vi "openDocuement.vi"(8 "error in (no error)":errorcluster, 11 "MS-Word in":refnum<class "MS-Word.lvclass">) -> (0 "error out":errorcluster, 3 "MS-Word out":refnum<class "MS-Word.lvclass">)   [LabVIEW 2017, in "LabVIEW NPOI.lvlib" / "MS-Word.lvclass"]
doc: "Protected dynamic dispatch method to open the <b>Document</b> file located at <b>File Path</b> for reading."
uses:
  MS-Word.lvclass
  C:/Users/Neo/Desktop/Dev_Tools_BR/LabVIEW_NPOI/src/LabVIEW NPOI/Document/Document.lvclass
  Document/Document.lvclass/Document.ctl
  MS-Word.lvclass/MS-Word.ctl
  Document/Get FilePath.vi
  xwpfDocument/xwpfDocument.lvclass
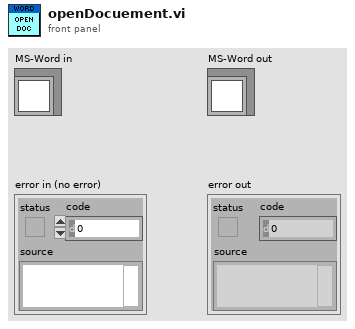
[diagram p1: front panel]
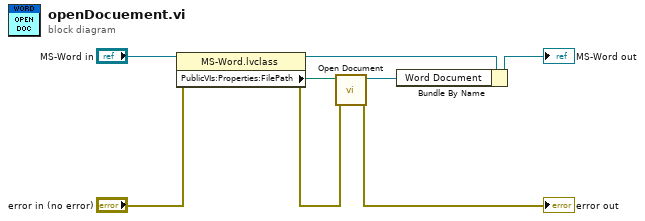
[diagram p0: block diagram]
diagram:
  n1 = property class="MS-Word.lvclass"(reference="MS-Word in", error in="error in (no error)") -> (reference out=w6:refnum<class "MS-Word.lvclass">, error out=w2:errorcluster, "PublicVIs:Properties:FilePath"=w5:path)
  n2 = call "Open Document.vi"("error in (no error)"=w2, "Document Path"=w5) -> ("error out"=→"error out":errorcluster, "xwpfDocument out"=w3:refnum<class "xwpfDocument.lvclass">)  [unwired: 8 in]
  n3 = Bundle By Name(cluster=w6, "Word Document"=w3) -> (→"MS-Word out":refnum<class "MS-Word.lvclass">)
